vi "query Starting and Num RB.vi"(8 "error in (no error)":errorcluster, 10 "RB Setting Param":T1, 11 "NR in":refnum<class "NR.lvclass">) -> (0 "error out":errorcluster, 2 "RB Value (0~273)":i32, 3 "NR out":refnum<class "NR.lvclass">)   [LabVIEW 2023, in "ANRITSU Call Box.lvlib" / "NR.lvclass"]
uses:
  NR.lvclass
  Type Definition/NR RB Setting Params for query.ctl
  NR.lvclass/NR.ctl
  ANRITSU Call Box.lvlib
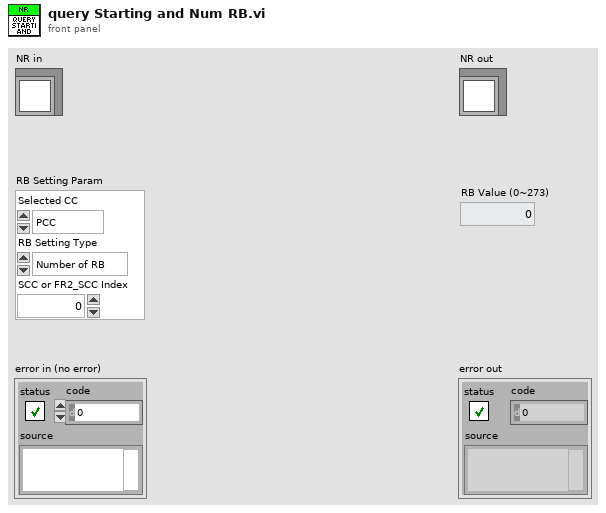
[diagram p1: front panel]
types:
  T1 = typedef "ANRITSU Call Box.lvlib/NR RB Setting Params for query.ctl" = cluster{"Selected CC":enum16{"PCC", "SCC", "FR2_PCC", "FR2_SCC"}, "RB Setting Type":enum16{"Number of RB", "Starting RB"}, "SCC or FR2_SCC Index":u32}
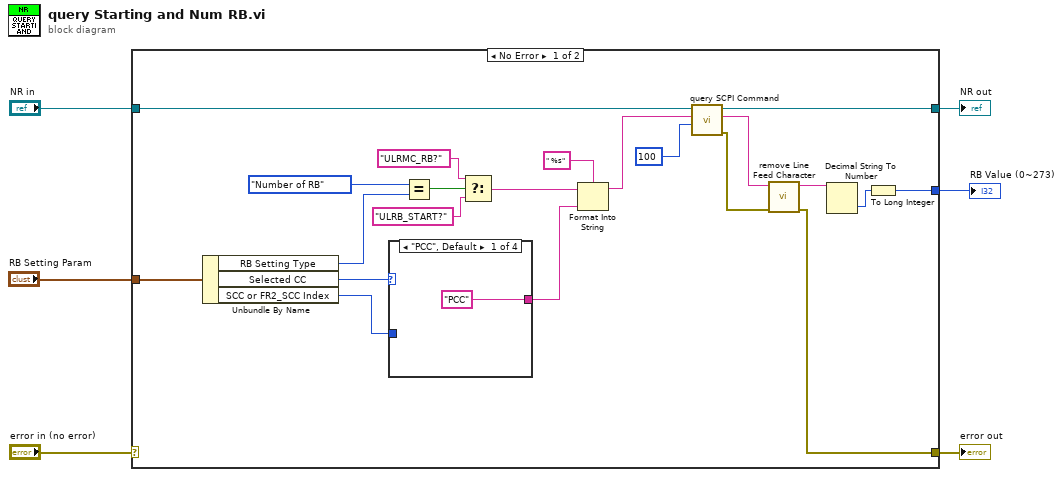
[diagram p0: block diagram]
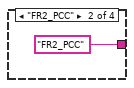
[diagram p2: hidden frame]
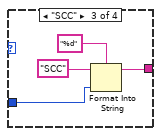
[diagram p3: hidden frame]
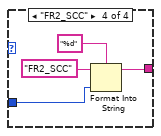
[diagram p4: hidden frame]
diagram:
  n1 = case shown="No Error" "error in (no error)" {
    selector: "error in (no error)" -> [_ w39]
    tunnel: [w8 w39] -> w5
    tunnel: [w14 w38] -> w3
    tunnel: "NR in" -> [w17 w38]
    tunnel: "RB Setting Param" -> [w27 _]
    tunnel: [w9 _] -> w1
    frame No Error {
      n2 = Unbundle By Name(w27) -> ("RB Setting Type"=w20:enum16{"Number of RB", "Starting RB"}, "Selected CC"=w26:enum16{"PCC", "SCC", "FR2_PCC", "FR2_SCC"}, "SCC or FR2_SCC Index"=w25:u32)
      n3 = case shown="\"PCC\", Default" w26 {
        tunnel: w25 -> [_ _ w30 w34]
        tunnel: ["PCC" "FR2_PCC" w31 w35] -> w18
        frame "PCC", Default {
        }
        frame "FR2_PCC" {
        }
        frame "SCC" {
          n4 = Format Into String(format string="%d", initial string="SCC", w30) -> (resulting string=w31:string)  [unwired: 1 in, 1 out]
        }
        frame "FR2_SCC" {
          n5 = Format Into String(format string="%d", initial string="FR2_SCC", w34) -> (resulting string=w35:string)  [unwired: 1 in, 1 out]
        }
      }
      n6 = Equal?(x=enum16{"Number of RB", "Starting RB"}."Number of RB", y=w20) -> (x = y?=w23:bool)
      n7 = Select(t="ULRMC_RB?" ("format string"), s=w23, f="ULRB_START?" ("format string")) -> (s? t:f=w19:string)
      n8 = Format Into String(format string=" %s", initial string=w19, w18) -> (resulting string=w16:string)  [unwired: 1 in, 1 out]
      n9 = call "query SCPI Command.vi"("Read Buffer Length"=u32 100, "SCPI Command"=w16, "NR in"=w17) -> ("error out"=w12:errorcluster, "Read Buffer String"=w13:string, "NR out"=w14:refnum<class "NR.lvclass">)  [unwired: 6 in]
      n10 = call "remove Line Feed Character.vi"("error in"=w12, "Query String"=w13) -> ("error out"=w8:errorcluster, "Line Feed Removed String"=w10:string)  [unwired: 8 in]
      n11 = Decimal String To Number(string=w10) -> (number=w11:i32)  [unwired: 2 in, 1 out]
      n12 = To Long Integer(number=w11) -> (32bit integer=w9:i32)
    }
    frame Error {
    }
  }
  "error out" <- w5
  "NR out" <- w3
  "RB Value (0~273)" <- w1
